vi "Load Test Case from File.vi"(8 "error in":errorcluster, 9 "Test Class Path":path) -> (0 "error out":errorcluster, 1 "Test Case":refnum<class>[](array[class]))   [LabVIEW 2013, in "VITesterUtilities.lvlib"]
uses:
  Libraries/VITesterUtilities.lvlib
panel:
  # "Copyright © 2007 James Kring, Inc. All rights reserved.\n\nAuthor: Omar Mussa [omar.mussa@jameskring.com]\n\nThis library is provided \"AS IS\" ,WITHOUT WARRANTIES OR \nCONDITIONS OF ANY KIND, either express or implied.\n\nJames Kring, Inc. -- http://www.jameskring.com"
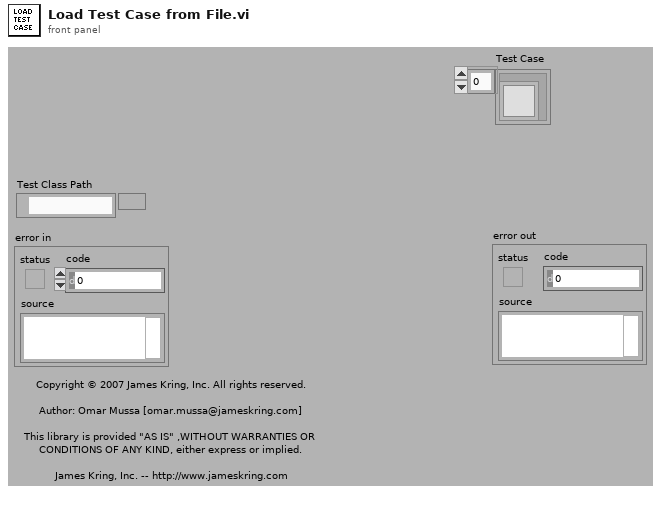
[diagram p1: front panel]
types:
  T1 = enum32{"invalid app kind", "Development System", "Run Time System", "Student Edition", "Embedded LabVIEW", "Evaluation", "Custom"}
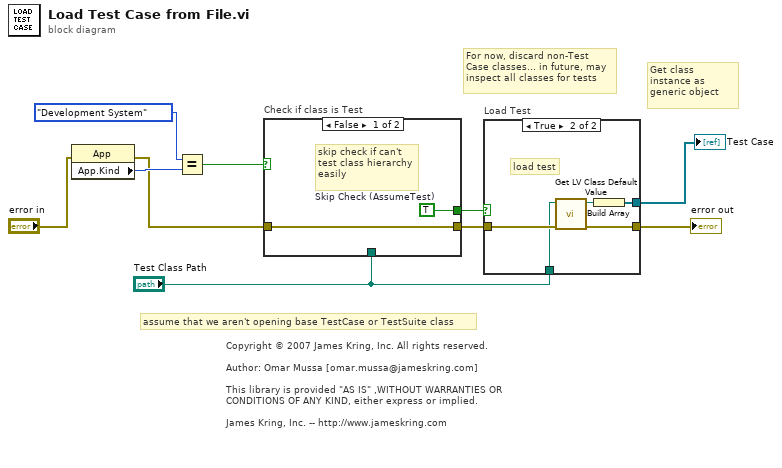
[diagram p0: block diagram]
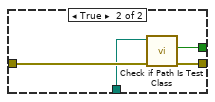
[diagram p2: hidden frame]
diagram:
  # "assume that we aren't opening base TestCase or TestSuite class"
  # "Get class instance as generic object"
  # "Copyright © 2007 James Kring, Inc. All rights reserved.\n\nAuthor: Omar Mussa [omar.mussa@jameskring.com]\n\nThis library is provided \"AS IS\" ,WITHOUT WARRANTIES OR \nCONDITIONS OF ANY KIND, either express or implied.\n\nJames Kring, Inc. -- http://www.jameskring.com"
  # "For now, discard non-Test Case classes... in future, may inspect all classes for tests"
  n1 = property class="App"(error in="error in") -> (error out=w2:errorcluster, "App.Kind"=w6:T1)  [unwired: 1 in, 1 out]
  n2 = Equal?(x=T1."Development System" ("y"), y=w6) -> (x = y?=w5:bool)
  n3 = case "Check if class is Test" shown="False" w5 {
    tunnel: w2 -> [w11 w16]
    tunnel: [w11 w15] -> w10
    tunnel: "Test Class Path" -> [_ w14]
    tunnel: [w12 w13] -> w7
    frame False {
      w12 = TRUE  # Skip Check (AssumeTest)
      # "skip check if can't\ntest class hierarchy\neasily"
    }
    frame True {
      n4 = call "Check if Path Is Test Class.vi"("error in"=w16, "Test Class Path"=w14) -> ("error out"=w15:errorcluster, "IsTestObject"=w13:bool)  [unwired: 7 in, 1 out]
    }
  }
  n5 = case "Load Test" shown="True" w7 {
    tunnel: w10 -> [w17 w22]
    tunnel: [w17 w21] -> w9
    tunnel: "Test Class Path" -> [_ w20]
    tunnel: [_ w18] -> w1
    frame False {
      # "do not load non\ntest objects"
    }
    frame True {
      # "load test"
      n6 = call <vilib>:"Get LV Class Default Value.vi"("error in (no error)"=w22, "class path"=w20) -> ("error out"=w21:errorcluster, "object"=w19:refnum<class>)  [unwired: 8 in]
      n7 = Build Array(w19) -> (w18:refnum<class>[])
    }
  }
  "error out" <- w9
  "Test Case" <- w1
